vi "is valid channel_extract_priv_method.vi"(11 "property names":string[](array[string])) -> (3 "Valid Channel":bool)   [LabVIEW 2020, in "Nominal-TDMS-Upload.lvlib" / "Nominal-TDMS-Upload.lvclass"]
uses:
  Nominal-TDMS-Upload.lvclass
  <vilib>/Nominal/Nominal IO Client/lv_src/Nominal Client/Nominal Client.lvclass
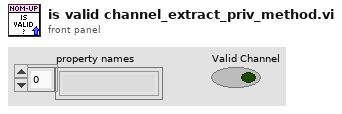
[diagram p1: front panel]
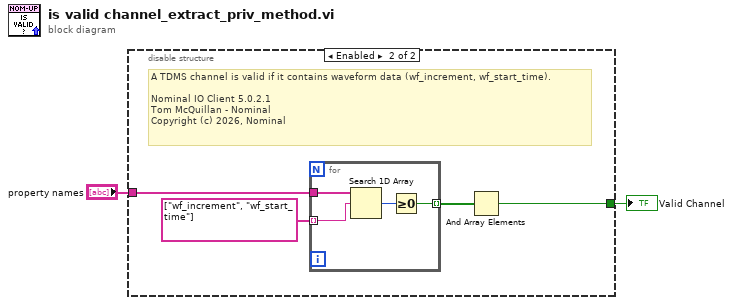
[diagram p0: block diagram]
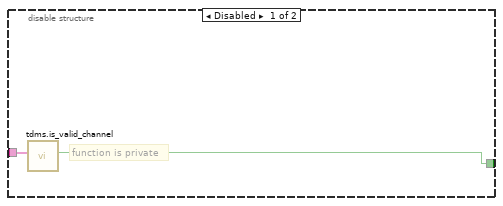
[diagram p2: hidden frame]
diagram:
  n1 = disable-structure shown="Enabled" {
    disable-tunnel: [w4 w6] -> w1
    disable-tunnel: "property names" -> [w3 w5]
    frame Disabled {
      # "function is private"
      n2 = call <vilib>:"tdms.is_valid_channel.vi"("TDMS Property Names"=w3) -> ("Valid Channel"=w4:bool)  [unwired: 10 in]
    }
    frame Enabled {
      # "A TDMS channel is valid if it contains waveform data (wf_increment, wf_start_time).\n\nNominal IO Client 5.0.2.1\nTom McQuillan - Nominal\nCopyright (c) 2026, Nominal"
      n3 = for {
        tunnel: w5 -> [w12]
        tunnel: string[] ["wf_increment", "wf_start_time"] ("element") -> [w11] mode=indexing
        tunnel: [w9] -> w7 mode=indexing
        n4 = Search 1D Array(1D array=w12, element=w11) -> (index of element=w10:i32)  [unwired: 1 in]
        n5 = Greater Or Equal To 0?(x=w10) -> (x >= 0?=w9:bool)
      }
      n6 = And Array Elements(Boolean array=w7) -> (logical AND=w6:bool)
    }
  }
  "Valid Channel" <- w1
